vi "ASD Base info.vi"(6 "error in":errorcluster, 11 "Base Table":T4(array[cluster]) {"Value 3" format="%.2g"}) -> (0 "Base N info":T1, 3 "B Cluster":T2, 4 "error out":errorcluster)   [LabVIEW 2018]
panel:
  out "Color IDX":u32[](array[numeric])
  out "Base ex Composition":string[](array[string])
  out "STD S Level [pA]":dbl[](array[numeric])
  out "Base IDX":i32[](array[numeric])
  out "Base S Level":dbl[](array[numeric])
  out "Base Composition":string[](array[string])
  out "B cluster":T3 {"Value 3" format="%.2g"}
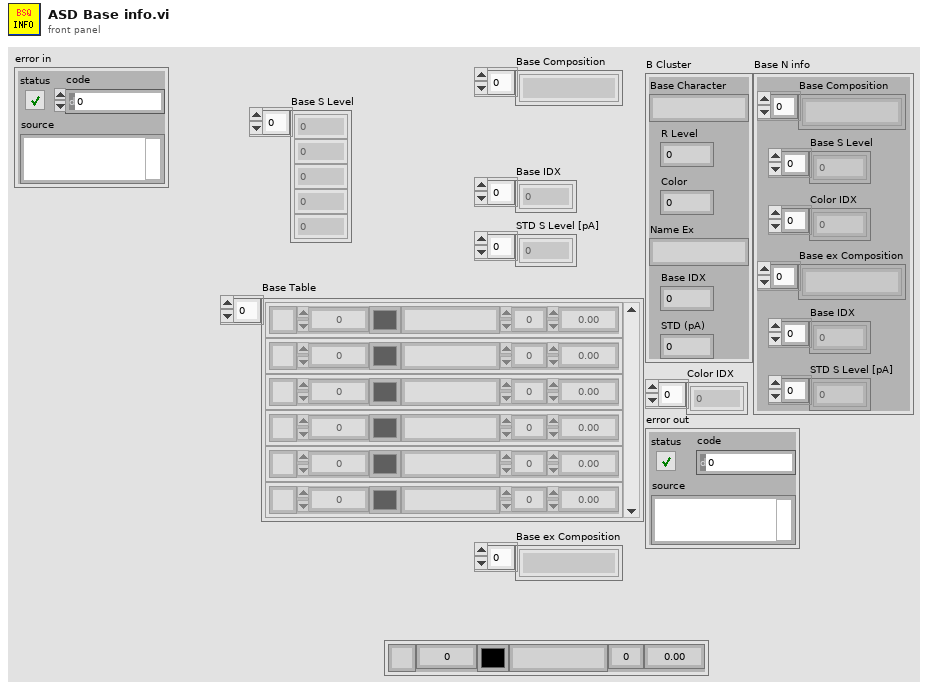
[diagram p1: front panel]
types:
  T1 = cluster{"Base Composition":string[], "Base S Level":dbl[], "Color IDX":u32[], "Base ex Composition":string[], "Base IDX":i32[], "STD S Level [pA]":dbl[]}
  T2 = cluster{"Base Character":string, "R Level":dbl, "Color":u32, "Name Ex":string, "Base IDX":dbl, "STD (pA)":dbl}
  T3 = cluster{"Name":string, "Value":dbl, "Color":u32, "Name 2":string, "Value 2":dbl, "Value 3":dbl}
  T4 = cluster{"Name":string, "Value":dbl, "Color":u32, "Name 2":string, "Value 2":i32, "Value 3":dbl}[]
  T5 = cluster{"Name":string, "Value":dbl, "Color":u32, "Name 2":string, "Value 2":i32, "Value 3":dbl}
  T6 = cluster{string[], dbl[], u32[], string[], i32[], dbl[]}
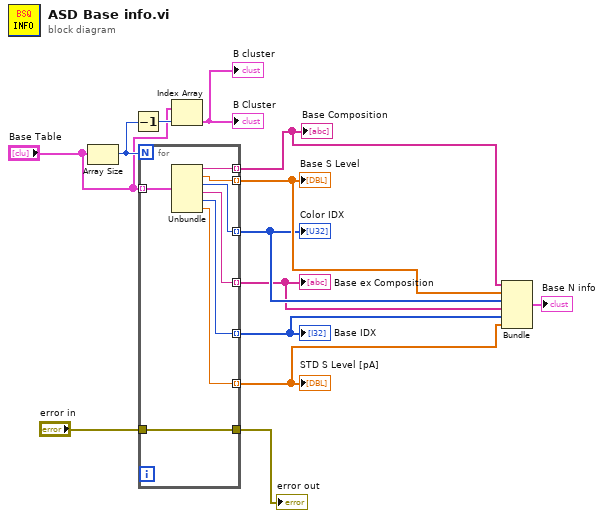
[diagram p0: block diagram]
diagram:
  n1 = Array Size(array="Base Table") -> (size(s)=w11:i32)
  n2 = Decrement(x=w11) -> (x-1=w13:i32)
  n3 = for {
    N: w11 -> [_]
    tunnel: "Base Table" -> [w21] mode=indexing
    tunnel: [w20] -> w8 mode=indexing
    tunnel: [w19] -> w7 mode=indexing
    tunnel: [w18] -> w6 mode=indexing
    tunnel: [w17] -> w5 mode=indexing
    tunnel: [w16] -> w4 mode=indexing
    tunnel: [w15] -> w3 mode=indexing
    tunnel: "error in" -> [w14]
    tunnel: [w14] -> w1
    n4 = Unbundle(w21) -> ("Name"=w20:string, "Value"=w19:dbl, "Color"=w18:u32, "Name 2"=w17:string, "Value 2"=w16:i32, "Value 3"=w15:dbl)
  }
  "Base Composition" <- w8
  "Base S Level" <- w7
  "Base IDX" <- w4
  "STD S Level [pA]" <- w3
  "Base ex Composition" <- w5
  "Color IDX" <- w6
  "error out" <- w1
  n5 = Index Array(array="Base Table", index=w13) -> (element=→"B cluster" →"B Cluster":T5)
  n6 = Bundle(w8, w7, w6, w5, w4, w3) -> (→"Base N info":T6)  [unwired: 1 in]
